vi "Load_Hardware_Config.vi"(8 "error in (no error)":errorcluster) -> (0 "error out":errorcluster, 3 "Device Context Cluster":T1)   [LabVIEW 2021]
doc: "This VI load from hardware configution file the device parameters and configuration"
uses:
  subVIs/Device Context/Device Context Cluster.ctl
  Motor/Motor.lvclass
  Elevator/Elevator.lvclass
  Modbus_Master/Modbus_Master.lvclass
  ServoDrive/ServoDrive.lvclass
  Modbus_RTU/Modbus_RTU.lvclass
  C:/Users/lincoln.lucio/Documents/Lincoln/Documentos Pessoais/meus docs/Projetos pessoais/Projeto Sciranda/projeto_versioned/sciranda/Modbus_Master/Modbus_Master.lvclass
  Modbus_RTU/Modbus_RTU.lvclass/Modbus_RTU.ctl
  Modbus_TCP/Modbus_TCP.lvclass
  Modbus_TCP/Modbus_TCP.lvclass/Modbus_TCP.ctl
  Modbus_Master/Modbus_Master.lvclass/Modbus_Master.ctl
  Elevator/Elevator.lvclass/Elevator.ctl
  Motor/Motor.lvclass/Motor.ctl
  WEG_SCA06_Modbus/WEG_SCA06_Modbus.lvclass
  C:/Users/lincoln.lucio/Documents/Lincoln/Documentos Pessoais/meus docs/Projetos pessoais/Projeto Sciranda/projeto_versioned/sciranda/ServoDrive/ServoDrive.lvclass
  WEG_SCA06_Modbus/WEG_SCA06_Modbus.lvclass/WEG_SCA06_Modbus.ctl
  ServoDrive/ServoDrive.lvclass/ServoDrive.ctl
  Modbus_RTU/Accessor VIs/Write VISA resource name.vi
  Modbus_RTU/Accessor VIs/Write baud rate.vi
  Modbus_RTU/Accessor VIs/Write parity.vi
  Modbus_RTU/Accessor VIs/Write serial type.vi
  Modbus_TCP/Accessor VIs/Write Address.vi
  Modbus_TCP/Accessor VIs/Write Port.vi
  Modbus_Master/Accessor VIs/Write unit ID.vi
  Modbus_Master/Accessor VIs/Write Timeout(ms).vi
  WEG_SCA06_Modbus/Accessor VIs/Write Modbus_Master.lvclass.vi
  ServoDrive/Accessor VIs/Write Accel_ms_krpm.vi
  ServoDrive/Accessor VIs/Write Decel_ms_krpm.vi
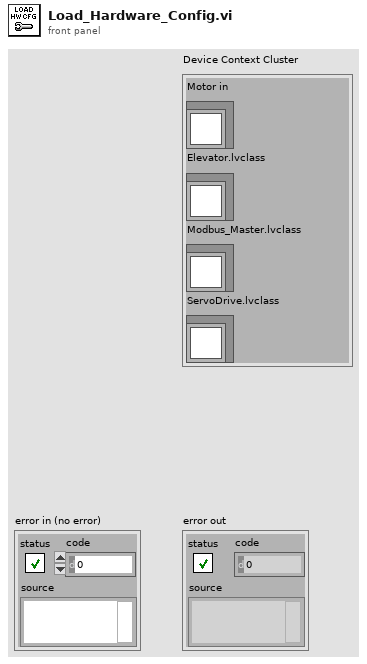
[diagram p1: front panel]
types:
  T1 = typedef "Device Context Cluster.ctl" = cluster{"Motor in":refnum<class "Motor.lvclass">, "Elevator.lvclass":refnum<class "Elevator.lvclass">, "Modbus_Master.lvclass":refnum<class "Modbus_Master.lvclass">, "ServoDrive.lvclass":refnum<class "ServoDrive.lvclass">}
  T2 = cluster{"AI_Channel":string, "AO_Channel":string}
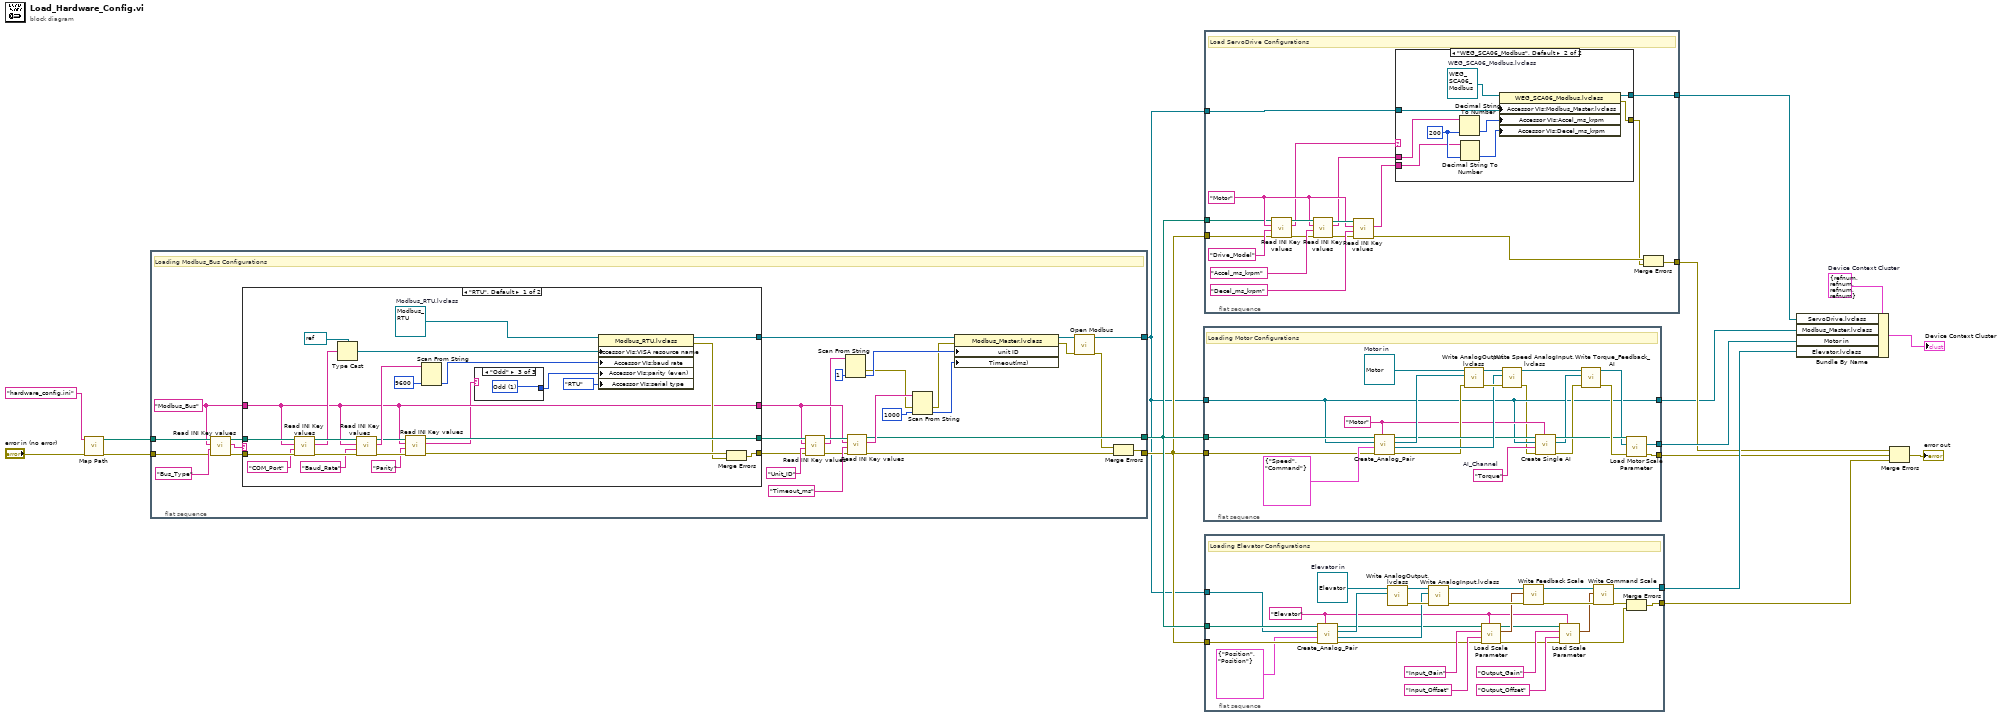
[diagram p0: block diagram]
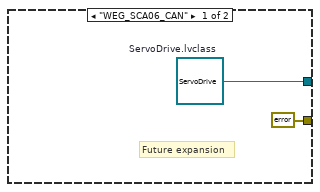
[diagram p2: hidden frame]
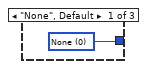
[diagram p3: hidden frame]
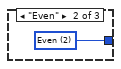
[diagram p4: hidden frame]
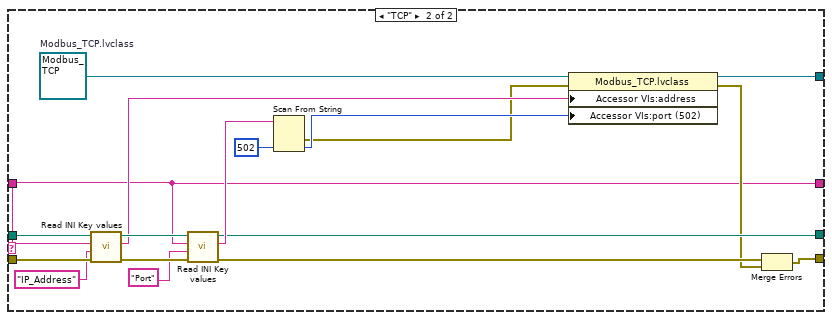
[diagram p5: hidden frame]
diagram:
  w13 = T1 {"Motor in"=refnum, "Elevator.lvclass"=refnum, "Modbus_Master.lvclass"=refnum, "ServoDrive.lvclass"=refnum}  # Device Context Cluster
  n1 = call "Map Path.vi"("error in (no error)"="error in (no error)", "file or folder path pattern"="hardware_config.ini" ("pattern")) -> ("error out"=w7:errorcluster, "Path Out"=w8:path)  [unwired: 8 in]
  n2 = flat-sequence {
    tunnel: w8 -> [w47]
    tunnel: w7 -> [w45]
    tunnel: [w22] -> w1
    tunnel: [w21] -> w6
    tunnel: [w18] -> w5
    frame #0 {
      w37 = "Modbus_Bus" ("section")
      # "Loading Modbus_Bus Configurations"
      n3 = call "Read INI Key values.vi"("error in (no error)"=w45, "key"="Bus_Type" ("section"), "section"=w37, "Path In"=w47) -> ("error out"=w38:errorcluster, "value"=w44:string, "Path Out"=w39:path)  [unwired: 5 in]
      n4 = case shown="\"RTU\", Default" w44 {
        tunnel: w39 -> [w72 w93]
        tunnel: w38 -> [w71 w92]
        tunnel: w37 -> [w50 w76]
        tunnel: [w68 w90] -> w34
        tunnel: [w52 w80] -> w35
        tunnel: [w54 w85] -> w36
        tunnel: [w50 w76] -> w33
        frame "RTU", Default {
          w69 = refnum<class "Modbus_RTU.lvclass"> refnum  # Modbus_RTU.lvclass
          n5 = call "Read INI Key values.vi"("error in (no error)"=w71, "key"="COM_Port", "section"=w50, "Path In"=w72) -> ("error out"=w66:errorcluster, "value"=w57:string, "Path Out"=w67:path)  [unwired: 5 in]
          n6 = Type Cast(type=refnum<visa-resource-name> refnum ("VISA resource name"), x=w57) -> (*(type *) &x=w56:refnum<visa-resource-name>)
          n7 = call "Read INI Key values.vi"("error in (no error)"=w66, "key"="Baud_Rate", "section"=w50, "Path In"=w67) -> ("error out"=w60:errorcluster, "value"=w63:string, "Path Out"=w61:path)  [unwired: 5 in]
          n8 = call "Read INI Key values.vi"("error in (no error)"=w60, "key"="Parity", "section"=w50, "Path In"=w61) -> ("error out"=w53:errorcluster, "value"=w49:string, "Path Out"=w54:path)  [unwired: 5 in]
          n9 = Scan From String(input string=w63, default 1=u32 9600 ("baud rate")) -> (output 1=w62:u32)  [unwired: 3 in, 3 out]
          n10 = case shown="\"Odd\"" w49 {
            tunnel: [w73 w74 w75] -> w48
            frame "None", Default {
              w73 = u16 0 items=["None", "Odd", "Even", "Mark", "Space"] ("parity (even)")
            }
            frame "Even" {
              w74 = u16 2 items=["None", "Odd", "Even", "Mark", "Space"] ("parity (even)")
            }
            frame "Odd" {
              w75 = u16 1 items=["None", "Odd", "Even", "Mark", "Space"] ("parity (even)")
            }
          }
          n11 = property class="Modbus_RTU.lvclass"(reference=w69, "Accessor VIs:VISA resource name"=w56, "Accessor VIs:baud rate"=w62, "Accessor VIs:parity (even)"=w48, "Accessor VIs:serial type"=enum16{"RTU", "ASCII"}."RTU" ("serial type")) -> (reference out=w68:refnum<class "Modbus_RTU.lvclass">, error out=w51:errorcluster)  [unwired: 1 in]
          n12 = Merge Errors(w53, w51) -> (w52:errorcluster)
        }
        frame "TCP" {
          w82 = refnum<class "Modbus_TCP.lvclass"> refnum  # Modbus_TCP.lvclass
          n13 = call "Read INI Key values.vi"("error in (no error)"=w92, "key"="IP_Address", "section"=w76, "Path In"=w93) -> ("error out"=w88:errorcluster, "value"=w83:string, "Path Out"=w89:path)  [unwired: 5 in]
          n14 = call "Read INI Key values.vi"("error in (no error)"=w88, "key"="Port", "section"=w76, "Path In"=w89) -> ("error out"=w84:errorcluster, "value"=w86:string, "Path Out"=w85:path)  [unwired: 5 in]
          n15 = Scan From String(input string=w86, default 1=u16 502 ("port (502)")) -> (error out=w78:errorcluster, output 1=w79:u16)  [unwired: 3 in, 2 out]
          n16 = property class="Modbus_TCP.lvclass"(reference=w82, error in=w78, "Accessor VIs:address"=w83, "Accessor VIs:port (502)"=w79) -> (reference out=w90:refnum<class "Modbus_TCP.lvclass">, error out=w77:errorcluster)
          n17 = Merge Errors(w84, w77) -> (w80:errorcluster)
        }
      }
      n18 = call "Read INI Key values.vi"("error in (no error)"=w35, "key"="Unit_ID", "section"=w33, "Path In"=w36) -> ("error out"=w40:errorcluster, "value"=w28:string, "Path Out"=w41:path)  [unwired: 5 in]
      n19 = Scan From String(input string=w28, default 1=u8 1 ("unit ID")) -> (error out=w25:errorcluster, output 1=w29:u8)  [unwired: 3 in, 2 out]
      n20 = call "Read INI Key values.vi"("error in (no error)"=w40, "key"="Timeout_ms", "section"=w33, "Path In"=w41) -> ("error out"=w19:errorcluster, "value"=w26:string, "Path Out"=w21:path)  [unwired: 5 in]
      n21 = Scan From String(input string=w26, error in=w25, default 1=1000 ("Timeout(ms)")) -> (error out=w24:errorcluster, output 1=w23:i32)  [unwired: 2 in, 2 out]
      n22 = property class="Modbus_Master.lvclass"(reference=w34, error in=w24, "unit ID"=w29, "Timeout(ms)"=w23) -> (reference out=w32:refnum<class "Modbus_Master.lvclass">, error out=w31:errorcluster)
      n23 = call-dynamic "Open Modbus.vi"("error in (no error)"=w31, "Modbus_Master in"=w32) -> ("error out"=w20:errorcluster, "Modbus_Master out"=w22:refnum<class "Modbus_Master.lvclass">)  [unwired: 8 in]
      n24 = Merge Errors(w20, w19) -> (w18:errorcluster)
    }
  }
  n25 = flat-sequence {
    tunnel: [w109] -> w10
    tunnel: [w108] -> w9
    tunnel: w6 -> [w100]
    tunnel: w5 -> [w99]
    tunnel: w1 -> [w95]
    tunnel: [w95] -> w2
    frame #0 {
      w98 = "Torque"  # AI_Channel
      w113 = refnum<class "Motor.lvclass"> refnum  # Motor in
      w96 = "Motor" ("section")
      # "Loading Motor Configurations"
      n26 = call "Create_Analog_Pair.vi"("section"=w96, "error in (no error)"=w99, "Analog Pair Key"=T2 {"AI_Channel"="Speed", "AO_Channel"="Command"}, "Modbus_Master.lvclass"=w95, "Config File in"=w100) -> ("error out"=w101:errorcluster, "AnalogInput.lvclass"=w110:refnum<class "AnalogInput.lvclass">, "AnalogOutput.lvclass"=w111:refnum<class "AnalogOutput.lvclass">, "Config File Out"=w105:path)  [unwired: 3 in]
      n27 = call "Write AnalogOutput.lvclass.vi"("error in (no error)"=w101, "AnalogOutput.lvclass"=w111, "Motor in"=w113) -> ("error out"=w112:errorcluster, "Motor out"=w114:refnum<class "Motor.lvclass">)  [unwired: 7 in]
      n28 = call "Write Speed AnalogInput.lvclass.vi"("error in (no error)"=w112, "AnalogInput.lvclass"=w110, "Motor in"=w114) -> ("error out"=w94:errorcluster, "Motor out"=w107:refnum<class "Motor.lvclass">)  [unwired: 7 in]
      n29 = call "Create Single AI.vi"("section"=w96, "error in (no error)"=w94, "AI_Channel"=w98, "Modbus_Master.lvclass"=w95, "Path In"=w105) -> ("error out"=w103:errorcluster, "AnalogInput.lvclass"=w102:refnum<class "AnalogInput.lvclass">, "Path Out"=w104:path)  [unwired: 4 in]
      n30 = call "Write Torque_Feedback_AI.vi"("error in (no error)"=w103, "AnalogInput.lvclass"=w102, "Motor in"=w107) -> ("error out"=w106:errorcluster, "Motor out"=w97:refnum<class "Motor.lvclass">)  [unwired: 7 in]
      n31 = call "Load Motor Scale Parameter.vi"("error in (no error)"=w106, "Motor in"=w97, "config file in"=w104) -> ("error out"=w109:errorcluster, "Motor out"=w108:refnum<class "Motor.lvclass">)  [unwired: 6 in, 1 out]
    }
  }
  n32 = flat-sequence {
    tunnel: [w124] -> w4
    tunnel: w6 -> [w123]
    tunnel: w5 -> [w122]
    tunnel: w1 -> [w121]
    tunnel: [w118] -> w3
    frame #0 {
      w126 = "Motor" ("key")
      # "Load ServoDrive Configurations"
      n33 = call "Read INI Key values.vi"("error in (no error)"=w122, "key"="Drive_Model", "section"=w126, "Path In"=w123) -> ("error out"=w130:errorcluster, "value"=w125:string, "Path Out"=w131:path)  [unwired: 5 in]
      n34 = call "Read INI Key values.vi"("error in (no error)"=w130, "key"="Accel_ms_krpm", "section"=w126, "Path In"=w131) -> ("error out"=w128:errorcluster, "value"=w117:string, "Path Out"=w127:path)  [unwired: 5 in]
      n35 = call "Read INI Key values.vi"("error in (no error)"=w128, "key"="Decel_ms_krpm", "section"=w126, "Path In"=w127) -> ("error out"=w120:errorcluster, "value"=w116:string)  [unwired: 5 in, 1 out]
      n36 = case shown="\"WEG_SCA06_Modbus\", Default" w125 {
        tunnel: [w135 w141] -> w124
        tunnel: w121 -> [_ w143]
        tunnel: [errorcluster {"status"=FALSE, "code"=0, "source"=""} ("error out") w142] -> w119
        tunnel: w117 -> [_ w140]
        tunnel: w116 -> [_ w137]
        frame "WEG_SCA06_CAN" {
          w135 = refnum<class "ServoDrive.lvclass"> refnum  # ServoDrive.lvclass
          # "Future expansion"
        }
        frame "WEG_SCA06_Modbus", Default {
          w138 = 200 ("Accel/Decel Default")
          w144 = refnum<class "WEG_SCA06_Modbus.lvclass"> refnum  # WEG_SCA06_Modbus.lvclass
          n37 = Decimal String To Number(string=w140, default (0L)=w138) -> (number=w139:i32)  [unwired: 1 in, 1 out]
          n38 = Decimal String To Number(string=w137, default (0L)=w138) -> (number=w136:i32)  [unwired: 1 in, 1 out]
          n39 = property class="WEG_SCA06_Modbus.lvclass"(reference=w144, "Accessor VIs:Modbus_Master.lvclass"=w143, "Accessor VIs:Accel_ms_krpm"=w139, "Accessor VIs:Decel_ms_krpm"=w136) -> (reference out=w141:refnum<class "WEG_SCA06_Modbus.lvclass">, error out=w142:errorcluster)  [unwired: 1 in]
        }
      }
      n40 = Merge Errors(w120, w119) -> (w118:errorcluster)
    }
  }
  n41 = flat-sequence {
    tunnel: [w146] -> w14
    tunnel: [w165] -> w12
    tunnel: w5 -> [w151]
    tunnel: w6 -> [w149]
    tunnel: w1 -> [w147]
    frame #0 {
      w172 = refnum<class "Elevator.lvclass"> refnum  # Elevator in
      w148 = "Elevator" ("section")
      # "Loading Elevator Configurations"
      n42 = call "Create_Analog_Pair.vi"("section"=w148, "error in (no error)"=w151, "Analog Pair Key"=T2 {"AI_Channel"="Position", "AO_Channel"="Position"}, "Modbus_Master.lvclass"=w147, "Config File in"=w149) -> ("error out"=w159:errorcluster, "AnalogInput.lvclass"=w162:refnum<class "AnalogInput.lvclass">, "AnalogOutput.lvclass"=w163:refnum<class "AnalogOutput.lvclass">, "Config File Out"=w158:path)  [unwired: 3 in]
      n43 = call "Write AnalogOutput.lvclass.vi"("AnalogOutput.lvclass"=w163, "Elevator in"=w172) -> ("error out"=w171:errorcluster, "Elevator out"=w170:refnum<class "Elevator.lvclass">)  [unwired: 8 in]
      n44 = call "Write AnalogInput.lvclass.vi"("error in (no error)"=w171, "AnalogInput.lvclass"=w162, "Elevator in"=w170) -> ("error out"=w169:errorcluster, "Elevator out"=w164:refnum<class "Elevator.lvclass">)  [unwired: 7 in]
      n45 = call "Load Scale Parameter.vi"("section"=w148, "error in (no error)"=w159, "Offset Key"="Input_Offset", "Gain Key"="Input_Gain", "config file in"=w158) -> ("error out"=w154:errorcluster, "Scale Parameters"=w157:cluster{"Gain":dbl, "Offset":dbl}, "config file out"=w153:path)  [unwired: 4 in]
      n46 = call "Write Feedback Scale.vi"("error in (no error)"=w169, "Feedback Scale"=w157, "Elevator in"=w164) -> ("error out"=w167:errorcluster, "Elevator out"=w168:refnum<class "Elevator.lvclass">)  [unwired: 7 in]
      n47 = call "Load Scale Parameter.vi"("section"=w148, "error in (no error)"=w154, "Offset Key"="Output_Offset", "Gain Key"="Output_Gain", "config file in"=w153) -> ("error out"=w145:errorcluster, "Scale Parameters"=w152:cluster{"Gain":dbl, "Offset":dbl})  [unwired: 4 in, 1 out]
      n48 = call "Write Command Scale.vi"("error in (no error)"=w167, "Command Scale"=w152, "Elevator in"=w168) -> ("error out"=w166:errorcluster, "Elevator out"=w165:refnum<class "Elevator.lvclass">)  [unwired: 7 in]
      n49 = Merge Errors(w166, w145) -> (w146:errorcluster)
    }
  }
  n50 = Bundle By Name(cluster=w13, "ServoDrive.lvclass"=w4, "Modbus_Master.lvclass"=w2, "Motor in"=w9, "Elevator.lvclass"=w12) -> (→"Device Context Cluster":T1)
  n51 = Merge Errors(w3, w10, w14) -> (→"error out":errorcluster)
